vi "API.vi"   [LabVIEW 2024]
uses:
  atsj peakcan basic.lvlib
  get parameter - u32.vi
  set parameter - u64.vi
  get channel handle - by bus channel index.vi
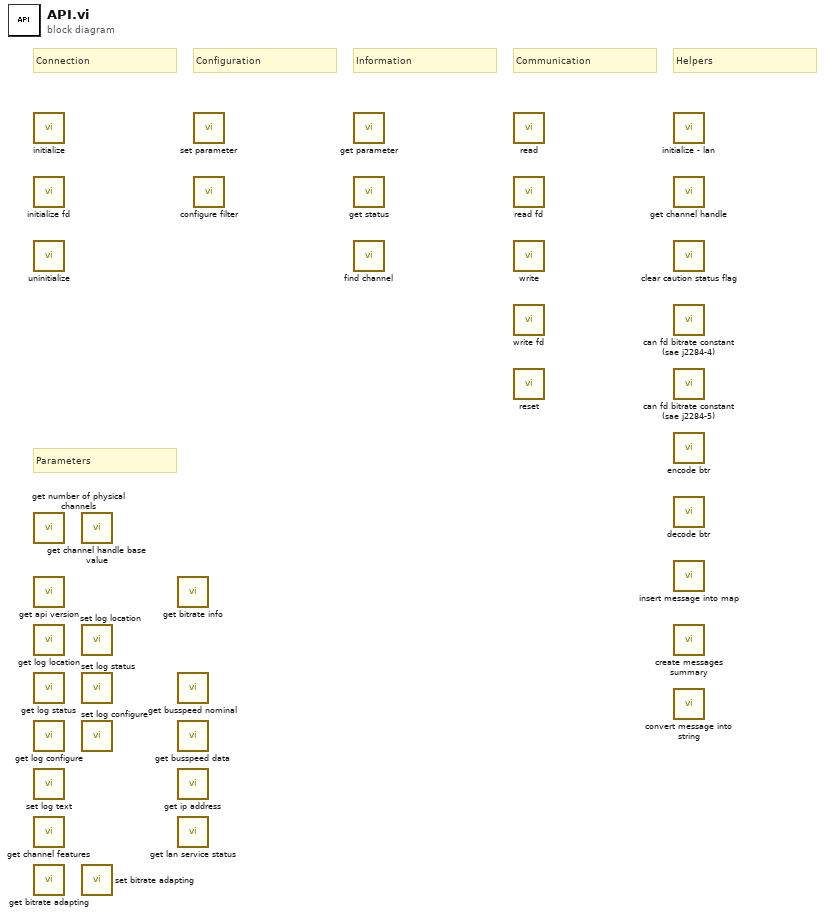
[diagram p0: block diagram]
diagram:
  # "Parameters"
  # "Helpers"
  # "Communication"
  # "Information"
  # "Configuration"
  # "Connection"
  n1 = call "initialize.vi"() -> ()  [unwired: 11 in, 1 out]
  n2 = call "initialize fd.vi"() -> ()  [unwired: 11 in, 1 out]
  n3 = call "uninitialize.vi"() -> ()  [unwired: 11 in, 1 out]
  n4 = call "get number of physical channels.vi"() -> ()  [unwired: 10 in, 2 out]
  n5 = call "get api version.vi"() -> ()  [unwired: 10 in, 2 out]
  n6 = call "get log location.vi"() -> ()  [unwired: 10 in, 2 out]
  n7 = call "get log status.vi"() -> ()  [unwired: 10 in, 2 out]
  n8 = call "get log configure.vi"() -> ()  [unwired: 9 in, 3 out]
  n9 = call "set log text.vi"() -> ()  [unwired: 11 in, 1 out]
  n10 = call "get channel features.vi"() -> ()  [unwired: 10 in, 2 out]
  n11 = call "get bitrate adapting.vi"() -> ()  [unwired: 10 in, 2 out]
  n12 = call "get channel handle base value.vi"() -> ()  [unwired: 10 in, 2 out]
  n13 = call "set log location.vi"() -> ()  [unwired: 11 in, 1 out]
  n14 = call "set log status.vi"() -> ()  [unwired: 11 in, 1 out]
  n15 = call "set log configure.vi"() -> ()  [unwired: 11 in, 1 out]
  n16 = call "set bitrate adapting.vi"() -> ()  [unwired: 11 in, 1 out]
  n17 = call "get bitrate info.vi"() -> ()  [unwired: 10 in, 2 out]
  n18 = call "get busspeed nominal.vi"() -> ()  [unwired: 10 in, 2 out]
  n19 = call "get busspeed data.vi"() -> ()  [unwired: 10 in, 2 out]
  n20 = call "get ip address.vi"() -> ()  [unwired: 10 in, 2 out]
  n21 = call "get lan service status.vi"() -> ()  [unwired: 10 in, 2 out]
  n22 = call-poly "set parameter.vi"() -> ()  [unwired: 11 in, 1 out]
  n23 = call "configure filter.vi"() -> ()  [unwired: 11 in, 1 out]
  n24 = call-poly "get parameter.vi"() -> ()  [unwired: 10 in, 2 out]
  n25 = call "get status.vi"() -> ()  [unwired: 9 in, 3 out]
  n26 = call "find channel.vi"() -> ()  [unwired: 10 in, 2 out]
  n27 = call "read.vi"() -> ()  [unwired: 8 in, 4 out]
  n28 = call "read fd.vi"() -> ()  [unwired: 8 in, 4 out]
  n29 = call "write.vi"() -> ()  [unwired: 11 in, 1 out]
  n30 = call "write fd.vi"() -> ()  [unwired: 11 in, 1 out]
  n31 = call "reset.vi"() -> ()  [unwired: 11 in, 1 out]
  n32 = call "initialize - lan.vi"() -> ()  [unwired: 10 in, 2 out]
  n33 = call-poly "get channel handle.vi"() -> ()  [unwired: 10 in, 2 out]
  n34 = call "clear caution status flag.vi"() -> ()  [unwired: 10 in, 2 out]
  n35 = call "can fd bitrate constant (sae j2284-4).vi"() -> ()  [unwired: 1 out]
  n36 = call "can fd bitrate constant (sae j2284-5).vi"() -> ()  [unwired: 1 out]
  n37 = call "encode btr.vi"() -> ()  [unwired: 11 in, 1 out]
  n38 = call "decode btr.vi"() -> ()  [unwired: 5 in, 7 out]
  n39 = call "insert message into map.vi"() -> ()  [unwired: 11 in, 1 out]
  n40 = call "create messages summary.vi"() -> ()  [unwired: 1 in, 1 out]
  n41 = call "convert message into string.vi"() -> ()  [unwired: 8 in, 4 out]
